vi "Example - MQTT performance test.vi"() -> ()   [LabVIEW 2019]
uses:
  src/KoRE-MQTT.lvlib
  src/KoRE-MQTT/Public/TypeDefs/MQTT Version.ctl
panel:
  out "Overlay":string
  in  "Topic Filters":T1(array[cluster])=[{"Topic"="#", "QoS"=enum."At most once"}]
  out "speed":cluster{dbl, u64}(graph)
  in  "stop":bool
  in  "Port":u16=1883
  in  "Host":string="test.mosquitto.org"
  in  "Password":string
  in  "Username":string
  in  "Version":T2=4 items=["3.11"=4, "5.0"=5]
  # "This VI will by default connect to the public test.mosquitto.org mqtt server and subscribe to all available topics. The maximum speed you see will probably be \nlimited by the output speed of the broker. In order to stress test or benchmark this client you should run your own mqtt broker and make sure you can generate\na lot of publish messages for this VI to be able to receive. The \"Example - Publish to localhost.vi\" is usefull if you have a local broker."
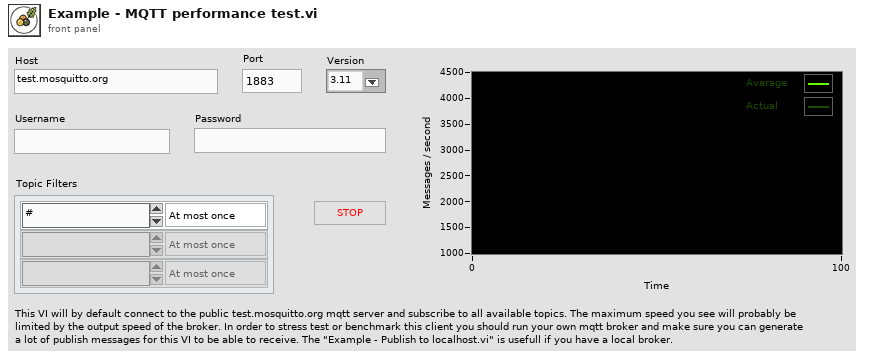
[diagram p1: front panel]
types:
  T1 = cluster{"Topic":string, "QoS":enum16{"At most once", "At least once", "Exactly once"}}[]
  T2 = typedef "KoRE-MQTT.lvlib/MQTT Version.ctl" = u8
  T3 = typedef "KoRE-MQTT.lvlib/MQTT Refnum.ctl" = refnum<vi>
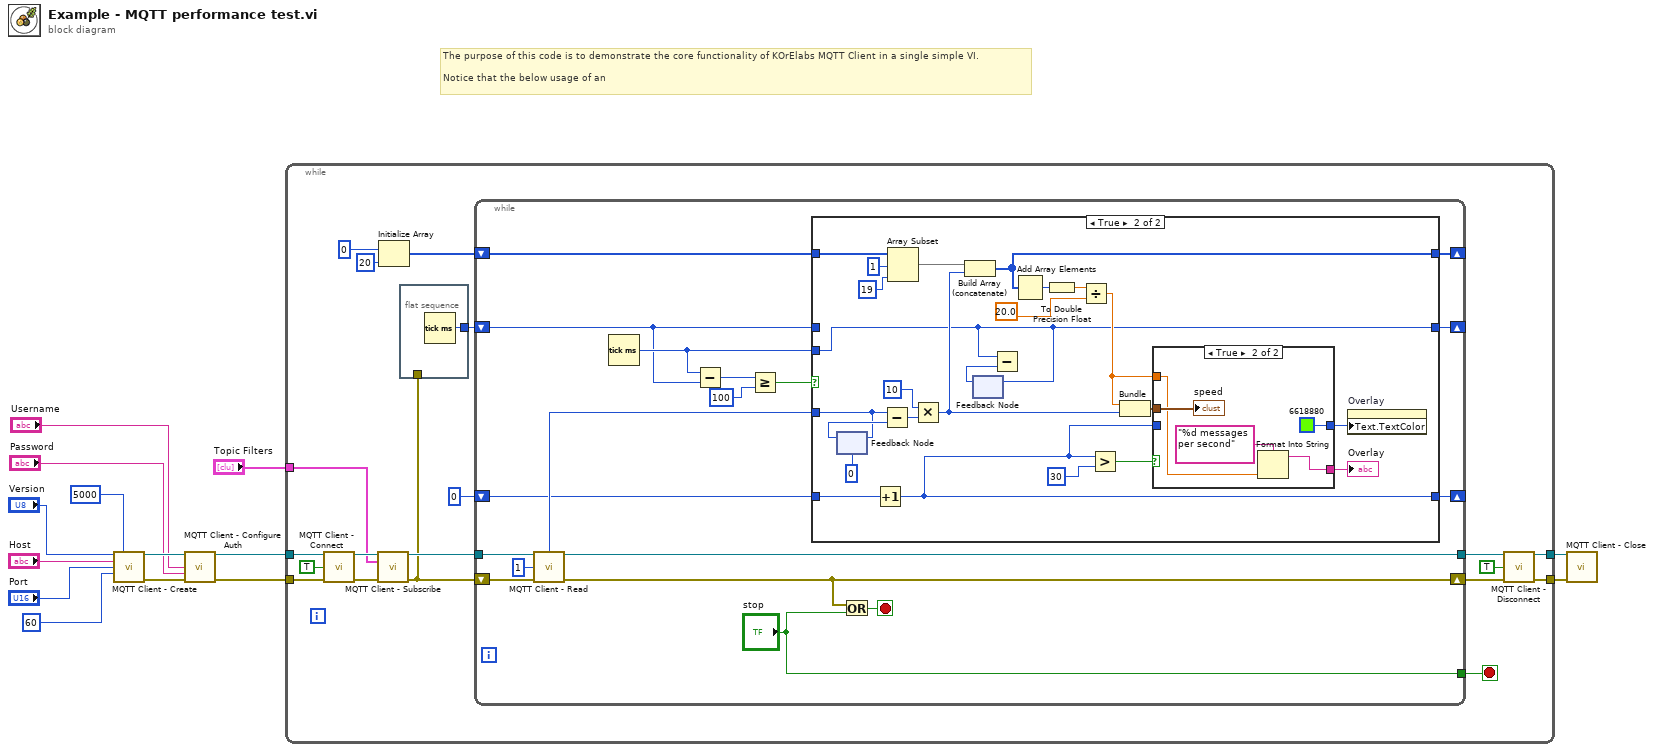
[diagram p0: block diagram]
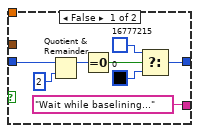
[diagram p3: hidden frame]
diagram:
  # "The purpose of this code is to demonstrate the core functionality of KOrElabs MQTT Client in a single simple VI.\n\nNotice that the below usage of an"
  n1 = call "MQTT Client - Create.vi"("Version (3.11)"="Version", "TCP Timeout (3000 ms)"=5000 ("TCP Timeout (ms)"), "Host (localhost)"="Host", "Port (1883)"="Port", "Keep Alive (60 s)"=u16 60 ("Keep Alive s (60)")) -> ("MQTT Session"=w12:T3, "error out"=w11:errorcluster)  [unwired: 9 in]
  n2 = call "MQTT Client - Configure Auth.vi"("MQTT Session"=w12, "Username"="Username", "Password"="Password", "error in (no error)"=w11) -> ("MQTT Session"=w3:T3, "error out"=w2:errorcluster)  [unwired: 10 in]
  n3 = while {
    tunnel: w2 -> [w31]
    tunnel: w3 -> [w30]
    tunnel: [w24] -> w14
    tunnel: [w22] -> w13
    tunnel: "Topic Filters" -> [w15]
    stop <- w27 stop-if-true
    n4 = call "MQTT Client - Connect.vi"("MQTT ref in"=w30, "Clean Start"=TRUE, "error in (no error)"=w31) -> ("mqtt ref"=w32:T3, "error out"=w33:errorcluster)  [unwired: 8 in, 3 out]
    n5 = call "MQTT Client - Subscribe.vi"("MQTT Session"=w32, "Multiple Topics"=w15, "error in (no error)"=w33) -> ("MQTT Session"=w29:T3, "error out"=w20:errorcluster)  [unwired: 11 in]
    n6 = Initialize Array(u64 0 ("speed"), 20 ("dimension size")) -> (w17:u64[])
    n7 = flat-sequence {
      tunnel: [w34] -> w21
      tunnel: w20 -> [_]
      frame #0 {
        n8 = Tick Count (ms)() -> (millisecond timer value=w34:u32)
      }
    }
    n9 = while {
      shift-right: [w50] -> w26
      shift-left: w20 -> [w52]
      tunnel: w29 -> [w51]
      tunnel: [w48] -> w25
      tunnel: ["stop"] -> w27
      shift-right: [w40] -> _
      shift-left: w21 -> [w39]
      shift-right: [w37] -> _
      shift-left: w17 -> [w38]
      shift-right: [w36] -> _
      shift-left: 0 -> [w35]
      stop <- w49 stop-if-true
      n10 = call "MQTT Client - Read.vi"("MQTT_Q In"=w51, "timeout (global)"=1 ("ms wait if no data (10 )"), "error in (no error)"=w52) -> ("# received"=w43:u64, "MQTT_Q Out"=w48:T3, "error out"=w50:errorcluster)  [unwired: 6 in, 4 out]
      n11 = Tick Count (ms)() -> (millisecond timer value=w41:u32)
      n12 = Subtract(x=w41, y=w39) -> (x-y=w45:u32)
      n13 = Greater Or Equal?(x=w45, y=u32 100) -> (x >= y?=w42:bool)
      n14 = case shown="True" w42 {
        tunnel: w43 -> [_ w77]
        tunnel: w41 -> [_ w57]
        tunnel: [w55 w57] -> w40
        tunnel: w39 -> [w55 _]
        tunnel: w38 -> [w54 w74]
        tunnel: [w54 w69] -> w37
        tunnel: w35 -> [w53 w65]
        tunnel: [w53 w60] -> w36
        frame False {
        }
        frame True {
          n15 = feedback #1(u64 0 ("# received")) -> (w79:u64)
          n16 = feedback-in #1(w77) -> ()
          n17 = Increment(x=w65) -> (x+1=w60:i32)
          n18 = Subtract(x=w77, y=w79) -> (x-y=w78:u64)
          n19 = Array Subset(array=w74, index=1, length=19) -> (w72:u64[])
          n20 = Multiply(x=u64 10, y=w78) -> (x*y=w68:u64)
          n21 = Build Array (concatenate)(w72, w68) -> (w69:u64[])
          n22 = feedback #2() -> (w56:u32)  [unwired: 1 in]
          n23 = feedback-in #2(w57) -> ()
          n24 = Subtract(x=w57, y=w56) -> ()  [unwired: 1 out]
          n25 = Add Array Elements(numeric array=w69) -> (sum=w71:u64)
          n26 = To Double Precision Float(number=w71) -> (double precision float=w59:dbl)
          n27 = Divide(x=w59, y=20.0) -> (x/y=w58:dbl)
          n28 = Greater?(x=w60, y=30) -> (0:w63:bool)
          n29 = Bundle(w58, w68) -> (w67:cluster{dbl, u64})  [unwired: 1 in]
          n30 = case shown="True" w63 {
            tunnel: w67 -> [_ w92]
            tunnel: ["Wait while baselining..." w89] -> w62
            tunnel: [w81 u32 6618880 ("Text.Text Colors:Text Color")] -> w61
            tunnel: w60 -> [w85 _]
            tunnel: w58 -> [_ w88]
            frame False {
              n31 = Quotient & Remainder(x=w85, y=2) -> (x-y*floor(x/y)=w84:i32)  [unwired: 1 out]
              n32 = Equal To 0?(x=w84) -> (x = 0?=w83:bool)
              n33 = Select(t=u32 16777215 ("Text.Text Colors:Text Color"), s=w83, f=u32 0 ("Text.Text Colors:Text Color")) -> (s? t:f=w81:u32)
            }
            frame True {
              n34 = Format Into String(format string="%d messages per second", w88) -> (resulting string=w89:string)  [unwired: 2 in, 1 out]
              "speed" <- w92
            }
          }
          "Overlay" <- w62
          n35 = property on="Overlay" class="Str"("Text.TextColor"=w61) -> ()  [unwired: 2 in, 2 out]
        }
      }
      n36 = Or(x=w50, y="stop") -> (x .or. y?=w49:bool)
    }
    n37 = call "MQTT Client - Disconnect.vi"("MQTT ref"=w25, "With Will"=TRUE, "error in (no error)"=w26) -> ("MQTT ref"=w24:T3, "error out"=w22:errorcluster)  [unwired: 11 in]
  }
  n38 = call "MQTT Client - Close.vi"("MQTT ref"=w14, "error in (no error)"=w13) -> ()  [unwired: 13 in, 1 out]
